vi "VIH - VI Doc Editor - Get Control Icon for Tree.vi"(8 "error in":errorcluster, 11 "Ctl Refnum":refnum<vi>) -> (0 "error out":errorcluster, 1 "Indicator":bool, 2 "Icon":T1, 3 "dup Ctl Refnum":refnum<vi>, 4 "Data Type":variant)   [LabVIEW 2014]
doc: "::: VI Helpeks :::\nCopyright (c) 2000-2026 Konstantin Shifershteyn. All rights reserved."
uses:
  <vilib>/picture/picture.llb/imagedata.ctl
panel:
  # "VI Helpeks\nCopyright (c) 2012-2026 Konstantin Shifershteyn"
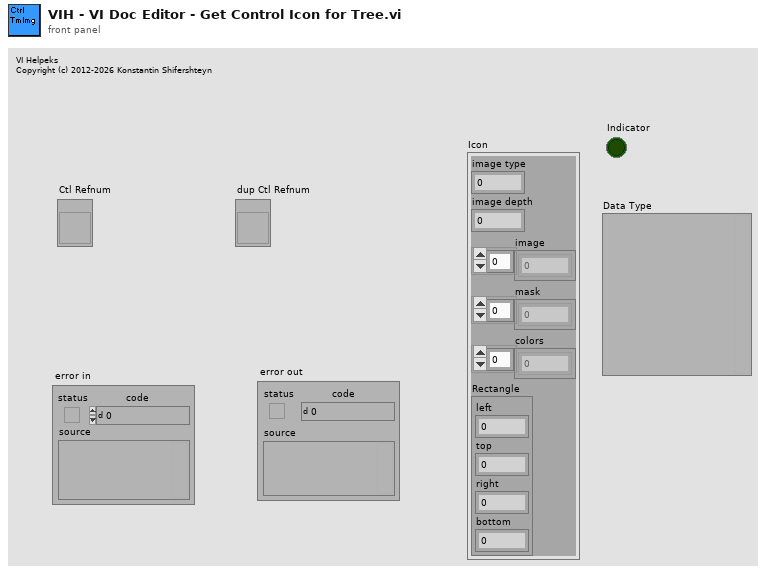
[diagram p1: front panel]
types:
  T1 = typedef "imagedata.ctl" = cluster{"image type":i32, "image depth":i32, "image":u8[], "mask":u8[], "colors":u32[], "Rectangle":cluster{"left":i16, "top":i16, "right":i16, "bottom":i16}}
  T2 = cluster{"left":i16, "top":i16, "right":i16, "bottom":i16}
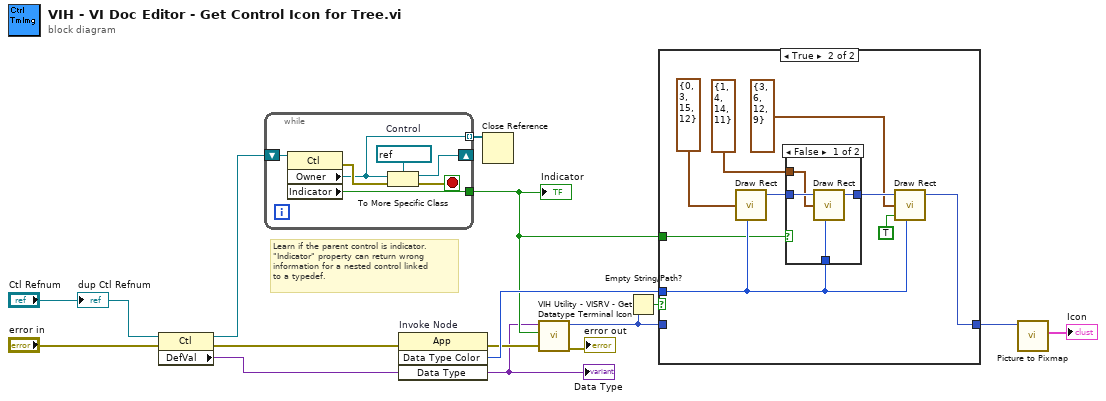
[diagram p0: block diagram]
diagram:
  # "Learn if the parent control is indicator.\n\"Indicator\" property can return wrong\ninformation for a nested control linked\nto a typedef."
  n1 = property class="Ctl"(reference="Ctl Refnum", error in="error in") -> (reference out=w9:refnum<vi>, error out=w8:errorcluster, "DefVal"=w4:variant)
  "Data Type" <- w4
  n2 = while {
    tunnel: [w18] -> w5
    shift-right: [w17] -> _
    shift-left: w9 -> [w19]
    tunnel: [w15] -> w14 mode=indexing
    stop <- w16 stop-if-true
    w20 = refnum<vi> refnum  # Control
    n3 = property class="Ctl"(reference=w19) -> (error out=w21:errorcluster, "Owner"=w15:refnum<vi>, "Indicator"=w18:bool)  [unwired: 1 in, 1 out]
    n4 = To More Specific Class(target class=w20, reference=w15, error in=w21) -> (specific class reference=w17:refnum<vi>, error out=w16:errorcluster)
  }
  "Indicator" <- w5
  n5 = invoke on="Invoke Node" class="App" method="Data Type Color"(error in=w8, "Data Type"=w4) -> (error out=w7:errorcluster, "Data Type Color"=w10:u32)  [unwired: 2 in, 2 out]
  n6 = Close Reference(reference=w14) -> ()  [unwired: 1 in, 1 out]
  n7 = call "VIH Utility - VISRV - Get Datatype Terminal Icon.vi"("error in"=w7, "Indicator"=w5, "Datatype"=w4) -> ("error out"=→"error out":errorcluster, "Icon"=w2:picture)  [unwired: 7 in]
  n8 = Empty String/Path?(string/path=w2) -> (empty?=w1:bool)
  n9 = case shown="True" w1 {
    tunnel: w10 -> [_ w31]
    tunnel: w5 -> [_ w24]
    tunnel: [w22 w23] -> w3
    tunnel: w2 -> [w22 _]
    frame False {
    }
    frame True {
      n10 = call <vilib>:"Draw Rect.vi"("rect"=T2 {"left"=0, "top"=3, "right"=15, "bottom"=12}, "color(black)"=w31) -> ("new picture"=w30:picture)  [unwired: 7 in]
      n11 = case shown="False" w24 {
        tunnel: w30 -> [w35 w36]
        tunnel: [w34 w36] -> w27
        tunnel: T2 {"left"=1, "top"=4, "right"=14, "bottom"=11} ("rect") -> [w33 _]
        tunnel: w31 -> [w32 _]
        frame False {
          n12 = call <vilib>:"Draw Rect.vi"("picture"=w35, "rect"=w33, "color(black)"=w32) -> ("new picture"=w34:picture)  [unwired: 6 in]
        }
        frame True {
        }
      }
      n13 = call <vilib>:"Draw Rect.vi"("picture"=w27, "rect"=T2 {"left"=3, "top"=6, "right"=12, "bottom"=9}, "fill?(F)"=TRUE, "color(black)"=w31) -> ("new picture"=w23:picture)  [unwired: 5 in]
    }
  }
  n14 = call <vilib>:"Picture to Pixmap.vi"("picture"=w3) -> ("image data"=→"Icon":T1)  [unwired: 9 in, 1 out]
  "dup Ctl Refnum" <- "Ctl Refnum"
